vi "Get Key Values.vi"(10 "Search Key":string, 11 "Configure Cluster":T1) -> (2 "Found?":bool, 3 "value":string)   [LabVIEW 2021]
uses:
  TypeDefs/Device Settings.ctl
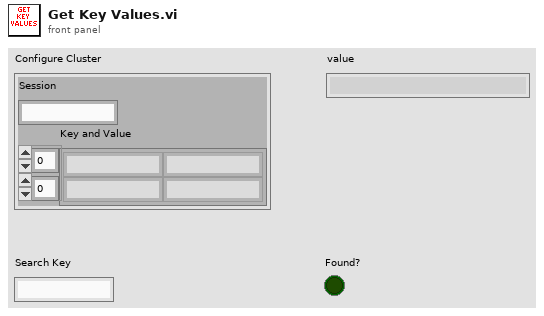
[diagram p1: front panel]
types:
  T1 = typedef "Device Settings.ctl" = cluster{"Session":string, "Key and Value":string[][]}
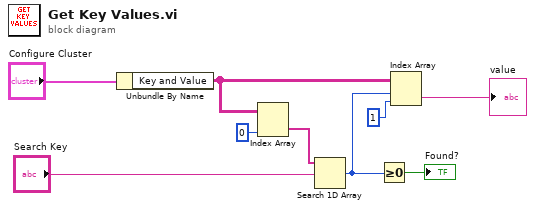
[diagram p0: block diagram]
diagram:
  n1 = Unbundle By Name("Configure Cluster") -> ("Key and Value"=w7:string[][])
  n2 = Index Array(array=w7, index (col)=0 ("disabled index (col)")) -> (element=w5:string[])  [unwired: 1 in]
  n3 = Search 1D Array(1D array=w5, element="Search Key") -> (index of element=w2:i32)  [unwired: 1 in]
  n4 = Greater Or Equal To 0?(x=w2) -> (x >= 0?=→"Found?":bool)
  n5 = Index Array(array=w7, index (row)=w2, index (col)=1 ("disabled index (col)")) -> (element=→"value":string)
